vi "Alter the IP Address of a protocol.vi"() -> ()   [LabVIEW 2020]
uses:
  <vilib>/addons/VeriStand Custom Device Scripting APIs/Instrument Addon/Libraries Directory/Protocols.lvlibp/TCP/TCP Settings.ctl
  <vilib>/addons/VeriStand Custom Device Scripting APIs/Instrument Addon/API/Custom Device/TCP Factory.vi
  <vilib>/addons/VeriStand Custom Device Scripting APIs/Instrument Addon/API/Custom Device/AK TCP Factory.vi
  <vilib>/addons/VeriStand Custom Device Scripting APIs/Instrument Addon/API/Instrument Addon Scripting API.lvlib
  <vilib>/addons/VeriStand Custom Device Scripting APIs/Instrument Addon/Libraries Directory/Protocols.lvlibp/TCP/TCP.lvclass
panel:
  in  "IP Address":string="10.0.0.10"
  in  "Output System Definition File":path=path "System Definition Files/Altered IP Address.nivssdf"
  in  "Input System Definition File":path=path "System Definition Files/Base with TCP.nivssdf"
  # "Overview: Alters the IP Address of a protocol while leaving other properties unchanged.\n\nThe VI executes the following steps:\n1. Uses the input refnum to fetch the protocol of the Instrument Addon Custom Device.\n2. Determines if the protocol is TCP or AK TCP.\n3. Alters the IP Address and inputs the new value to the appropriate protocol factory.\n4. Save System Definition file at the specification location.\n\nNote: The factory produces a protocol object that is used as an input for the Set Protocol node.\n\nInstructions:\n1. Browse to the system definition file to be used as input.\n2. Browse to a path to save the system definition file as output. This may be the same as the input file.\n3. Input the desired IP Address to update in the configured system definition file.\n4. Run the VI and verify its results."
  # "System Definition Files"
  # "Configuration"
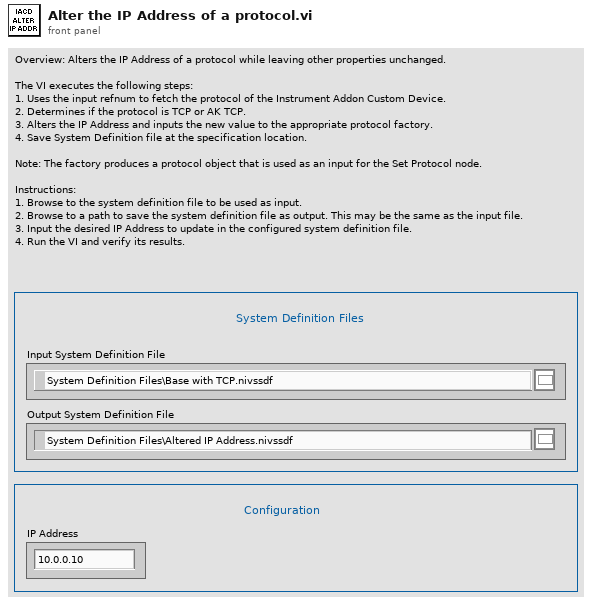
[diagram p1: front panel]
types:
  T1 = typedef "Protocols.lvlibp/TCP.lvclass/TCP Settings.ctl" = cluster{"IP Address":string, "Port":u16}
  T2 = typedef "Custom Device API.lvlib/Custom Device Item Ref.ctl" = u64
  T3 = typedef "Protocols.lvlibp/Protocol Parent.lvclass/Protocol Type.ctl" = enum16{"RS-XXX", "AK RS-XXX", "VISA", "TCPIP", "AK TCPIP", "UDP", "GPIB ConvBox"}
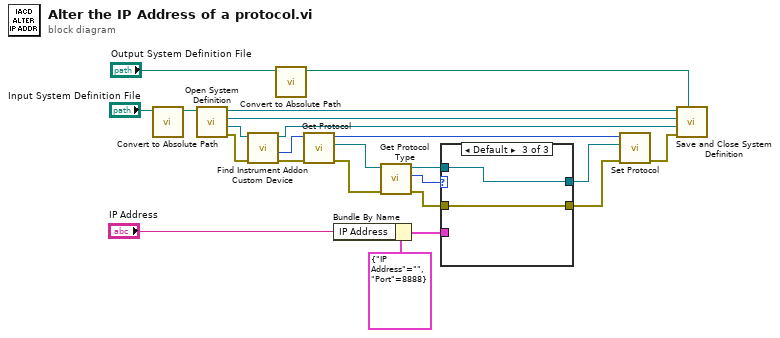
[diagram p0: block diagram]
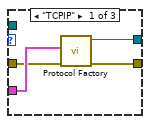
[diagram p2: hidden frame]
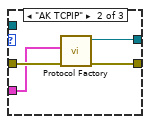
[diagram p3: hidden frame]
diagram:
  n1 = call "Convert to Absolute Path.vi"("System Definition File"="Input System Definition File") -> ("Absolute Path"=w7:path)  [unwired: 10 in]
  n2 = call "Open System Definition.vi"("System Definition File"=w7) -> ("error out"=w11:errorcluster, "Target Refnum"=w10:refnum<k24>, "Root Refnum"=w4:refnum<k24>, "System Definition Refnum"=w3:refnum<k24>)  [unwired: 7 in]
  n3 = call "Find Instrument Addon Custom Device.vi"("error in"=w11, "target in"=w10) -> ("error out"=w8:errorcluster, "NodeID"=w9:u64, "target out"=w5:refnum<k24>)  [unwired: 7 in]
  n4 = call "Convert to Absolute Path.vi"("System Definition File"="Output System Definition File") -> ("Absolute Path"=w1:path)  [unwired: 10 in]
  n5 = call <vilib>:"Get Protocol.vi"("error in (no error)"=w8, "instrument addon refnum in"=w9) -> ("error out"=w21:errorcluster, "protocol"=w22:refnum<class "Protocol Parent.lvclass">, "instrument addon refnum out"=w14:T2)  [unwired: 7 in]
  n6 = Bundle By Name(cluster=T1 {"IP Address"="", "Port"=8888} ("TCP settings"), "IP Address"="IP Address") -> (w18:T1)
  n7 = call <vilib>:"Get Protocol Type.vi"("error in (no error)"=w21, "protocol  in"=w22) -> ("error out"=w17:errorcluster, "protocol type"=w20:T3, "protocol out"=w19:refnum<class "Protocol Parent.lvclass">)  [unwired: 7 in]
  n8 = case shown="Default" w20 {
    tunnel: w19 -> [_ _ w32]
    tunnel: w18 -> [w27 w28 _]
    tunnel: w17 -> [w26 w29 w33]
    tunnel: [w25 w30 w32] -> w16
    tunnel: [w24 w31 w33] -> w15
    frame "TCPIP" {
      n9 = call-poly <vilib>:"Protocol Factory.vi"("error in (no error)"=w26, "settings"=w27) -> ("error out"=w24:errorcluster, "protocol out"=w25:refnum<class "Protocol Parent.lvclass">)  [unwired: 8 in]
    }
    frame "AK TCPIP" {
      n10 = call-poly <vilib>:"Protocol Factory.vi"("error in (no error)"=w29, "settings"=w28) -> ("error out"=w31:errorcluster, "protocol out"=w30:refnum<class "Protocol Parent.lvclass">)  [unwired: 8 in]
    }
    frame Default {
    }
  }
  n11 = call <vilib>:"Set Protocol.vi"("error in (no error)"=w15, "protocol"=w16, "instrument addon refnum in"=w14) -> ("error out"=w6:errorcluster)  [unwired: 7 in, 1 out]
  n12 = call "Save and Close System Definition.vi"("System Definition Path"=w1, "error in (no error)"=w6, "Target Refnum"=w5, "Root Refnum"=w4, "System Definition Refnum"=w3) -> ()  [unwired: 6 in, 1 out]
